vi "lab1_cw4.vi"() -> ()   [LabVIEW 2026]
uses:
  <vilib>/Platform/TimedLoop/XDataNode/wakeup.ctl
  <vilib>/Platform/TimedLoop/XDataNode/XDNodeRunTimeDep.lvlib
  <vilib>/Platform/TimedLoop/XDataNode/nitl_modes.ctl
  <vilib>/Platform/TimedLoop/XDataNode/timing_clust.ctl
  <vilib>/platform/TimedLoop/XDataNode/XDataNode.xnode
  <vilib>/eio/EIONode/EIONode.xnode
  <vilib>/rvi/eio/common/nirviEmuTemplateMethod_errors.vi
panel:
  in  "N":i32
  in  "M":i32
  in  "D":i32
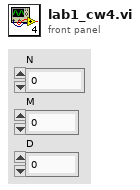
[diagram p1: front panel]
types:
  T1 = typedef "XDNodeRunTimeDep.lvlib/timing_clust.ctl" = cluster{"Expected End [f-1]":u64, "Actual End [f-1]":u64, "Finished Late? [f-1]":bool, "Expected End [i-1]":u64, "Actual End [i-1]":u64, "Finished Late? [i-1]":bool, "Expected Start [i]":u64, "Actual Start [i]":u64, "Expected Start [f]":u64, "Actual Start [f]":u64, "Source Name":string, "Structure Name":string, "Period":i64, "Deadline":i64, "Offset":i64, "Start":i64, "Priority":i32, "Timeout":i32, "Mode":T2, "Wakeup Reason":T3, "Error":errorcluster, "Source Type":string, "Secondary Source Type":string, "Global End Time":u64, "Global Start Time":u64, "Frame Duration":u64, "Iteration Duration":u64, "Assigned CPU":i32, "I/O Scan Engine Mode":u32}
  T2 = typedef "XDNodeRunTimeDep.lvlib/nitl_modes.ctl" = enum32{"No Change", "Process missed periods, maintain original phase", "Discard missed periods, maintain original phase", "Process missed periods, ignore original phase", "Discard missed periods, ignore original phase"}
  T3 = typedef "XDNodeRunTimeDep.lvlib/wakeup.ctl" = enum32{"Normal", "Aborted", "Asynchronous wakeup", "Timing source error", "Timed loop error", "Timeout"}
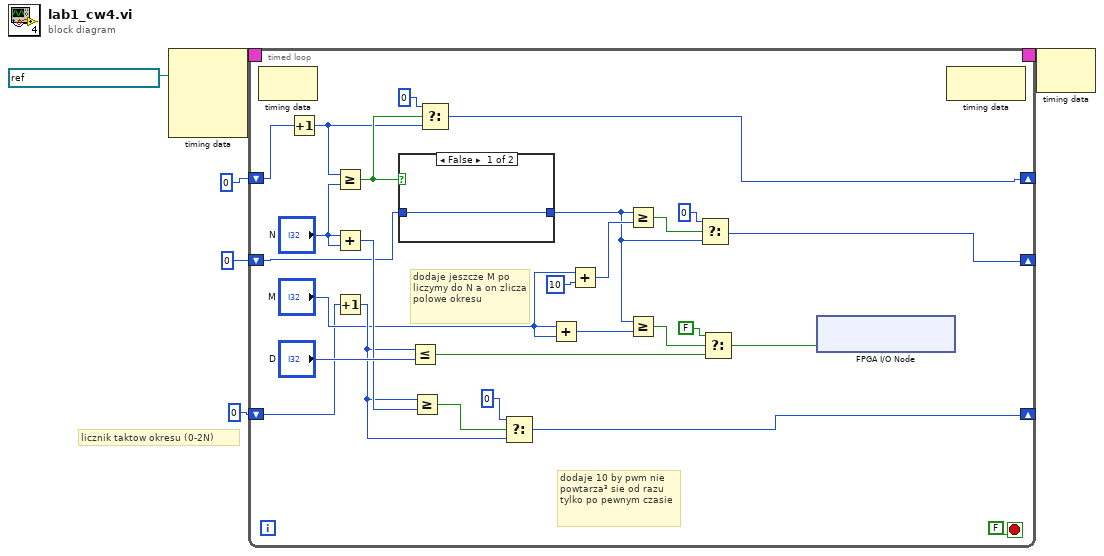
[diagram p0: block diagram]
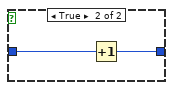
[diagram p2: hidden frame]
diagram:
  # "licznik taktow okresu (0-2N)"
  n1 = node-c288(refnum<k21> "40 MHz Onboard Clock" ("Source Name")) -> (w6:T1)  [unwired: 3 in]
  n2 = timed-loop {
    timing: w6 -> [_]
    timing-out: [_] -> w5
    shift-right: [w8] -> _
    shift-left: 0 -> [w13]
    shift-right: [w9] -> _
    shift-left: 0 -> [w12]
    shift-right: [w10] -> _
    shift-left: 0 -> [w11]
    stop <- FALSE stop-if-true
    # "dodaje 10 by pwm nie powtarza³ sie od razu tylko po pewnym czasie"
    # "dodaje jeszcze M po liczymy do N a on zlicza polowe okresu"
    n3 = node-c288() -> ()  [unwired: 1 in, 1 out]
    n4 = Increment(x=w13) -> (x+1=w22:i32)
    n5 = Greater Or Equal?(x=w22, y="N") -> (x >= y?=w29:bool)
    n6 = Add(x="N", y="N") -> (x+y=w19:i32)
    n7 = Increment(x=w11) -> (x+1=w17:i32)
    n8 = case shown="False" w29 {
      tunnel: w12 -> [w34 w35]
      tunnel: [w34 w36] -> w25
      frame False {
      }
      frame True {
        n9 = Increment(x=w35) -> (x+1=w36:i32)
      }
    }
    n10 = Less Or Equal?(x=w17, y="D") -> (x <= y?=w23:bool)
    n11 = Greater Or Equal?(x=w17, y=w19) -> (x >= y?=w18:bool)
    n12 = Select(t=0, s=w29, f=w22) -> (s? t:f=w8:i32)
    n13 = Select(t=0, s=w18, f=w17) -> (s? t:f=w10:i32)
    n14 = Add(x="M", y="M") -> (x+y=w14:i32)
    n15 = Add(x="M", y=10) -> (x+y=w27:i32)
    n16 = Greater Or Equal?(x=w25, y=w27) -> (x >= y?=w26:bool)
    n17 = Greater Or Equal?(x=w25, y=w14) -> (x >= y?=w31:bool)
    n18 = Select(t=0, s=w26, f=w25) -> (s? t:f=w9:i32)
    n19 = Select(t=FALSE, s=w31, f=w23) -> (s? t:f=w7:bool)
    n20 = xnode "FPGA I/O Node"("ConnectorA/DIO1"=w7) -> ()  [unwired: 1 in, 1 out]
    n21 = node-c288() -> ()  [unwired: 1 in, 1 out]
  }
  n22 = node-c288(w5) -> ()  [unwired: 1 out]
